vi "Configure Channel.vi"(8 "error in (no error)":errorcluster, 10 "DAQmx Task In":refnum<k21>, 11 "DAQmxVoltageChannel in":refnum<class "VoltageInChannel.lvclass">) -> (0 "error out":errorcluster, 2 "DAQmx Task":refnum<k21>)   [LabVIEW 2020, in "VolatusDAQConfig.lvlib" / "VoltageInChannel.lvclass"]
uses:
  VoltageInChannel.lvclass
  C:/dev/lv20CE/relink/lv-volatus/VolatusConfig/VolatusConfigElement/VolatusConfigElement.lvclass
  C:/dev/lv20CE/relink/lv-volatus/VolatusConfig/Channel/Channel.lvclass
  VolatusConfig/VolatusConfigElement/VolatusConfigElement.lvclass/VolatusConfigElement.ctl
  VoltageInChannel.lvclass/VoltageInChannel.ctl
  VolatusConfig/VolatusConfigElement/Element.vi
  VolatusConfig/VolatusConfigElement/Lookup Child by Name.vi
  VolatusConfig/Channel/Channel Config.lvclass
  lv-cdm/CDM-Config/Config Element/Lookup Child by Name.vi
  lv-cdm/CDM-Config/Config Element/Value (String).vi
  <vilib>/DAQmx/create/channels.llb/DAQmx Create Channel (AI-Voltage-Basic).vi
  C:/dev/lv20CE/relink/lv-volatus/VolatusDAQConfig/DAQmxChannel/DAQmxChannel.lvclass
  C:/dev/lv20CE/relink/lv-volatus/VolatusConfig/Channel/Channel Config.lvclass
  C:/dev/lv20CE/relink/lv-volatus/VolatusDAQConfig/DAQmxVoltageChannel/VoltageInChannel.lvclass
  VolatusConfig/VolatusConfigElement/VolatusConfigElement.lvclass
  <resource>/objmgr/daqmx.rc
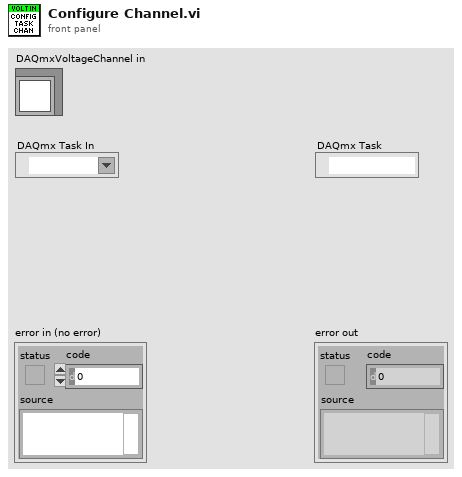
[diagram p1: front panel]
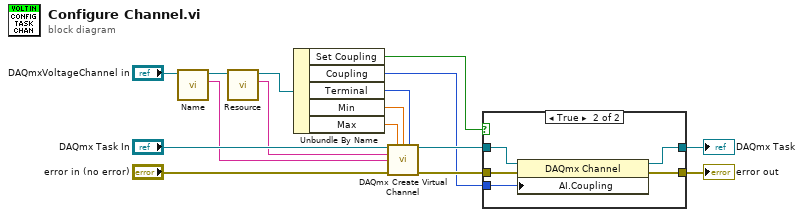
[diagram p0: block diagram]
diagram:
  n1 = call "Name.vi"("VolatusConfigElement in"="DAQmxVoltageChannel in") -> ("Name"=w7:string, "VolatusConfigElement out"=w8:refnum<class "VoltageInChannel.lvclass">)  [unwired: 8 in, 1 out]
  n2 = call "Resource.vi"("Channel in"=w8) -> ("Resource"=w9:string, "Channel out"=w10:refnum<class "VoltageInChannel.lvclass">)  [unwired: 8 in, 1 out]
  n3 = Unbundle By Name(w10) -> ("Set Coupling"=w2:bool, "Coupling"=w1:i32, "Terminal"=w13:i32, "Min"=w12:dbl, "Max"=w11:dbl)
  n4 = call-poly <vilib>:"DAQmx Create Virtual Channel.vi"("task in"="DAQmx Task In", "maximum value"=w11, "minimum value"=w12, "input terminal configuration"=w13, "physical channels"=w9, "name to assign"=w7, "error in"="error in (no error)") -> ("task out"=w5:refnum<k21>, "error out"=w6:errorcluster)  [unwired: 7 in]
  n5 = case shown="True" w2 {
    tunnel: w6 -> [w17 w23]
    tunnel: w5 -> [w18 w22]
    tunnel: [w18 w21] -> w4
    tunnel: [w17 w20] -> w3
    tunnel: w1 -> [_ w19]
    frame False {
    }
    frame True {
      n6 = property class="DAQmx Channel"(reference=w22, error in=w23, "AI.Coupling"=w19) -> (reference out=w21:refnum<k21>, error out=w20:errorcluster)
    }
  }
  "error out" <- w3
  "DAQmx Task" <- w4
